vi "Format Sample To Time.vi"(10 "Pitch (decimal) (1)":dbl=1.0, 11 "Samples":i32) -> (3 "Formatted Time":string)   [LabVIEW 2019, in "User Interface.lvlib"]
doc: "Convert the sample number into a time value in the form HH:MM:SS.s"
uses:
  User Interface.lvlib
  Packed Libraries/Globals.lvlibp/Constants.vi
  Packed Libraries/Globals.lvlibp
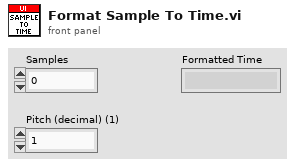
[diagram p1: front panel]
types:
  T1 = typedef "LVDateTimeRec.ctl" = cluster{"fractional second":dbl, "second":i32, "minute":i32, "hour":i32, "day of month":i32, "month":i32, "year":i32, "day of week":i32, "day of year":i32, "DST":i32}
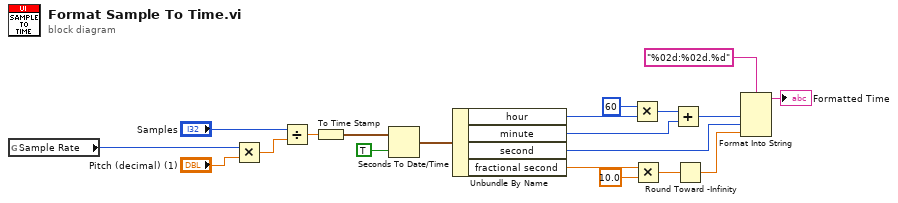
[diagram p0: block diagram]
diagram:
  n1 = global read "Constants.vi" "Sample Rate"() -> (w1:i32)
  n2 = Multiply(x=w1, y="Pitch (decimal) (1)") -> (x*y=w2:dbl)
  n3 = Divide(x="Samples", y=w2) -> (x/y=w19:dbl)
  n4 = To Time Stamp(1:w19) -> (0:w18:timestamp)
  n5 = Seconds To Date/Time(time stamp (now)=w18, to UTC (F)=TRUE) -> (date time rec=w16:T1)
  n6 = Unbundle By Name(w16) -> ("hour"=w14:i32, "minute"=w11:i32, "second"=w9:i32, "fractional second"=w8:dbl)
  n7 = Multiply(x=60, y=w14) -> (x*y=w12:i32)
  n8 = Multiply(x=w8, y=10.0) -> (x*y=w6:dbl)
  n9 = Add(x=w12, y=w11) -> (x+y=w10:i32)
  n10 = Round Toward -Infinity(1:w6) -> (0:w5:dbl)
  n11 = Format Into String(format string="%02d:%02d.%d", w10, w9, w5) -> (resulting string=→"Formatted Time":string)  [unwired: 2 in, 1 out]
